vi "Is Unicode.vi"(1 "Language":string) -> (0 "Is Unicode":bool)   [LabVIEW 2019, in "Language Selection.lvlib"]
doc: "- - -\nCopyright (c) 2026, Merecs Engineering GmbH"
uses:
  Language Selection.lvlib
panel:
  # "Connector Pane"
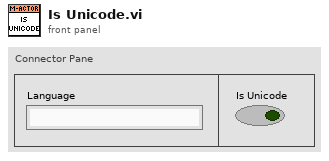
[diagram p1: front panel]
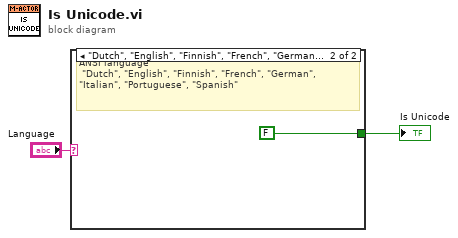
[diagram p0: block diagram]
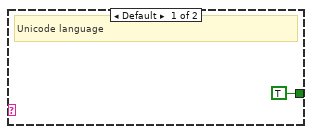
[diagram p2: hidden frame]
diagram:
  n1 = case shown="\"Dutch\", \"English\", \"Finnish\", \"French\", \"German\", \"Italian\", \"Portuguese\", \"Spanish\"" "Language" {
    tunnel: [TRUE FALSE] -> w2
    frame Default {
      # "Unicode language"
    }
    frame "Dutch", "English", "Finnish", "French", "German", "Italian", "Portuguese", "Spanish" {
      # "ANSI language\n \"Dutch\", \"English\", \"Finnish\", \"French\", \"German\", \"Italian\", \"Portuguese\", \"Spanish\""
    }
  }
  "Is Unicode" <- w2
